vi "Destroy Blackboard.vi"(8 "error in (no error)":errorcluster, 11 "Blackboard Reference":T1 {"refnum" format="%.0x"}) -> (0 "error out":errorcluster, 2 "readers_remaining":i32)   [LabVIEW 2021, in "Iceoryx.lvlib"]
uses:
  Iceoryx.lvlib
  SubVIs/Convert Error Core.vi
  Refnum/Typedef/BB Refnum.ctl
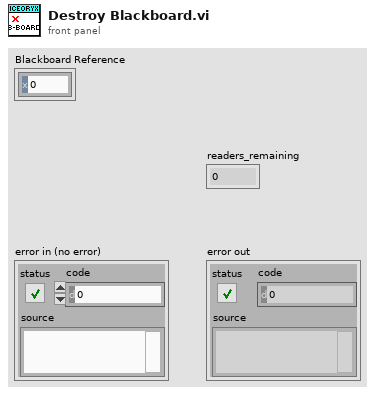
[diagram p1: front panel]
types:
  T1 = typedef "Iceoryx.lvlib/BB Refnum.ctl" = cluster{"refnum":u64, "BB":enum8{"bb"}}
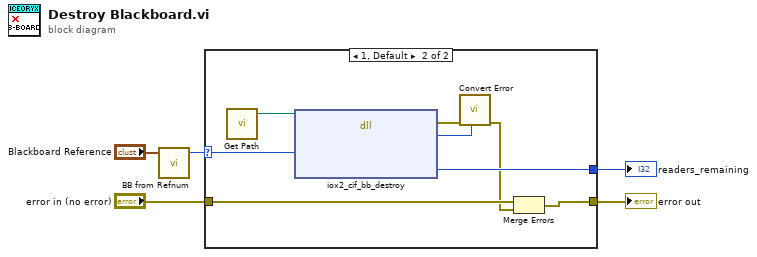
[diagram p0: block diagram]
diagram:
  n1 = call "BB from Refnum.vi"("BB Refnum"="Blackboard Reference") -> ("BB U64"=w1:u64)  [unwired: 4 in]
  n2 = case shown="1, Default" w1 {
    selector: w1 -> [_ w8]
    tunnel: [_ w14] -> w5
    tunnel: "error in (no error)" -> [w6 w11]
    tunnel: [w6 w9] -> w3
    frame 0 {
    }
    frame 1, Default {
      n3 = call "Get Path.vi"() -> ("libiox2_cif path"=w13:path)  [unwired: 4 in]
      n4 = dll-call lib="D:/dev/iceoryx2_lvwrapper/dist/iox2_cif.dll" fn="iox2_cif_bb_destroy"(path in=w13, "bb"=w8) -> (error out=w7:errorcluster, "return type"=w12:i32, "readers_remaining"=w14:i32)  [unwired: 4 in, 1 out]
      n5 = call "Convert Error.vi"("return type"=w12, "error in (no error)"=w7) -> ("error out"=w10:errorcluster)  [unwired: 9 in]
      n6 = Merge Errors(w11, w10) -> (w9:errorcluster)
    }
  }
  "error out" <- w3
  "readers_remaining" <- w5
